vi "validate.vi"(8 "error in":errorcluster, 11 "E2E Tag Exchange configuration in":refnum<class "E2E Tag Exchange configuration.lvclass">) -> (0 "error out":errorcluster, 3 "E2E Tag Exchange configuration out":refnum<class "E2E Tag Exchange configuration.lvclass">)   [LabVIEW 2015, in "E2E Tag Exchange configuration.lvclass"]
doc: "This function performs validation of the configuration. This function should be safe to call at any point and should not rely on anything in the runtime environment."
uses:
  E2E Tag Exchange configuration.lvclass
  E2E Tag Exchange configuration.lvclass/E2E Tag Exchange configuration.ctl
  <vilib>/NI/Tag Bus Module Framework/module configuration/TBM module configuration.lvclass
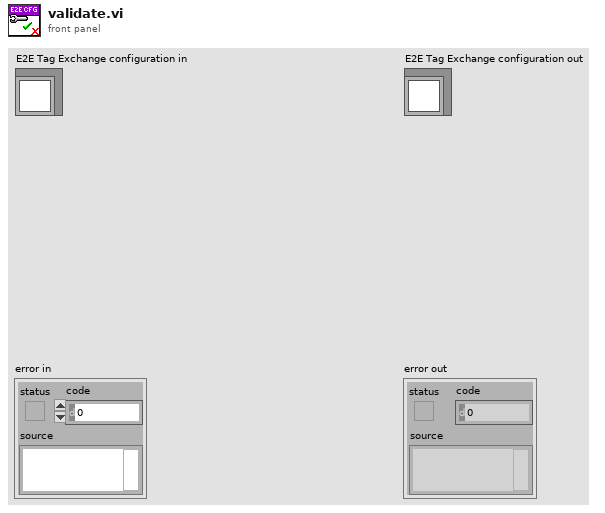
[diagram p1: front panel]
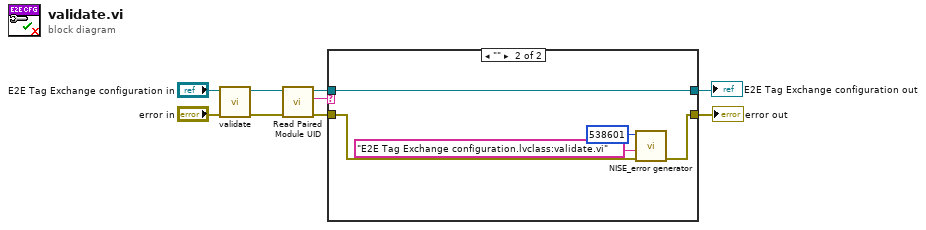
[diagram p0: block diagram]
diagram:
  n1 = call-parent "validate.vi"("error in"="error in", "configuration in"="E2E Tag Exchange configuration in") -> ("error out"=w6:errorcluster, "configuration out"=w7:refnum<class "E2E Tag Exchange configuration.lvclass">)  [unwired: 8 in]
  n2 = call "Read Paired Module UID.vi"("error in (no error)"=w6, "E2E Tag Exchange configuration in"=w7) -> ("error out"=w4:errorcluster, "Paired Module UID"=w5:string, "E2E Tag Exchange configuration out"=w3:refnum<class "E2E Tag Exchange configuration.lvclass">)  [unwired: 7 in]
  n3 = case shown="\"\"" w5 {
    tunnel: w4 -> [w10 w16]
    tunnel: w3 -> [w11 w15]
    tunnel: [w11 w15] -> w2
    tunnel: [w10 w14] -> w1
    frame Default {
    }
    frame "" {
      n4 = call <vilib>:"NISE_error generator.vi"("error in"=w16, "source"="E2E Tag Exchange configuration.lvclass:validate.vi", "error code (0)"=538601) -> ("error out"=w14:errorcluster)  [unwired: 6 in]
    }
  }
  "error out" <- w1
  "E2E Tag Exchange configuration out" <- w2
